vi "CallBack VI - OnActivated.vi"(4 "ActivationHandler":refnum<class "ActivationHandler.lvclass">, 5 "Event Data":cluster{"e":refnum<k24>}, 6 "Control Ref":refnum<k24>, 7 "Event Common Data":T1) -> ()   [LabVIEW 2026, in "ToastNotification.lvlib" / "ToastService.lvclass"]
doc: "Native OnActivated event callback, invoked by the .NET event registration. Borrow Event Data.e and Control Ref; never close these event-owned references. Convert the event data to LabVIEW Activation and release acquired temporary references before dynamically calling the injected ActivationHandler. The conversion error is passed to the handler error input. Last Callback Error is a diagnostic indicator, not an event queue or connector output. Keep handler work short."
uses:
  ToastService.lvclass
  C:/Users/loicw/Documents/LabVIEW/ToastNotifications/Sources/bins/Microsoft.Toolkit.Uwp.Notifications.dll
  bins/Microsoft.Toolkit.Uwp.Notifications.dll
  ActivationHandler/ActivationHandler.lvclass
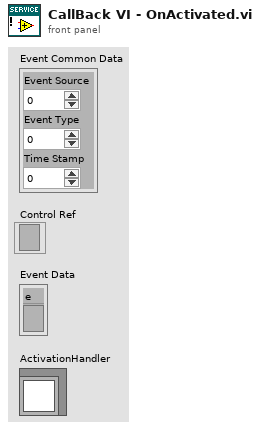
[diagram p1: front panel]
types:
  T1 = cluster{"Event Source":i32, "Event Type":u32, "Time Stamp":u32}
  T2 = typedef "ToastNotification.lvlib/Activation.ctl" = cluster{"Arguments":string, "User Inputs":T3[]}
  T3 = typedef "ToastNotification.lvlib/Argument.ctl" = cluster{"Key":string, "Value":string}
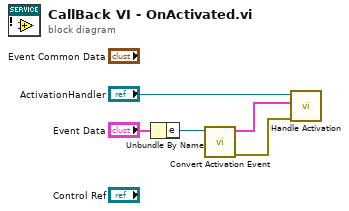
[diagram p0: block diagram]
diagram:
  n1 = Unbundle By Name("Event Data") -> ("e"=w3:refnum<k24>)
  n2 = call "Convert Activation Event.vi"("Activation Event Args"=w3) -> ("error out"=w2:errorcluster, "Activation"=w1:T2)  [unwired: 9 in]
  n3 = call-dynamic "Handle Activation.vi"("error in (no error)"=w2, "Activation"=w1, "ActivationHandler in"="ActivationHandler") -> ()  [unwired: 9 in]
